vi "TXT to TDMS.vi"(8 "error in":errorcluster caption="エラー入力（エラーなし）", 11 "Original File name (TXT)":path) -> (0 "error out":errorcluster caption="エラー出力", 3 "Raw data Graph":dbl[](graph))   [LabVIEW 2018]
uses:
  <vilib>/Utility/file.llb/Read Delimited Spreadsheet (DBL).vi
panel:
  out "file or folder exists?":bool caption="既存するファイルまたはフォルダ?"
  out "all rows":dbl[][](array[numeric]) format="%0.3f"
  out "Create File name (TDMS)":path
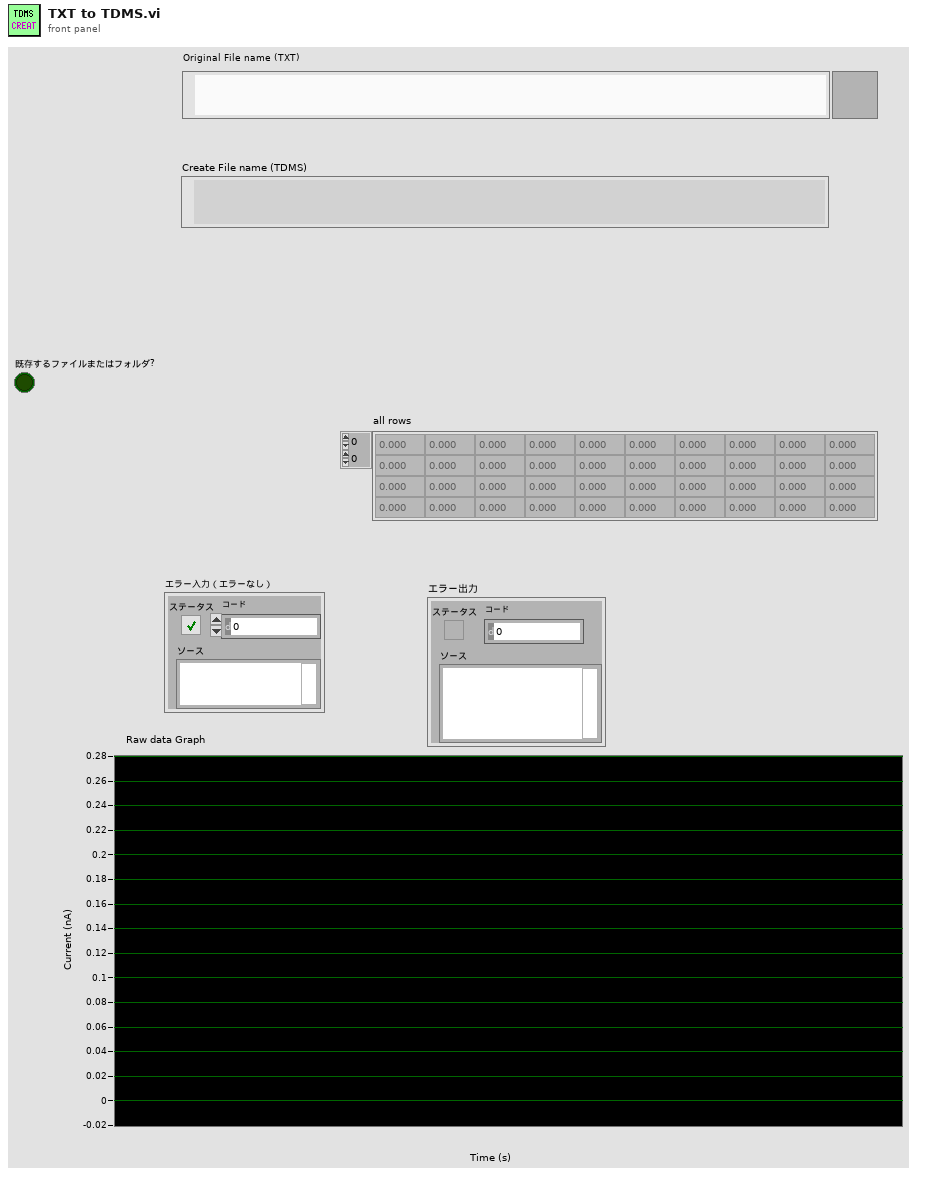
[diagram p1: front panel]
types:
  T1 = enum16{"open", "open or create", "create or replace", "create", "open (read-only)"}
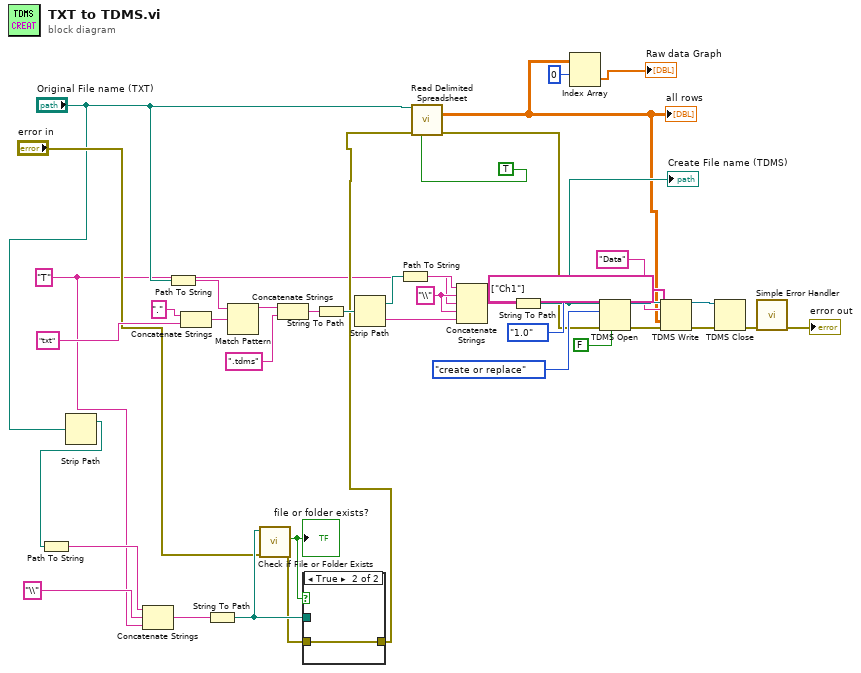
[diagram p0: block diagram]
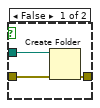
[diagram p2: hidden frame]
diagram:
  w4 = "T" ("Folder Name")
  w29 = "\\" ("文字列")
  n1 = Strip Path(path="Original File name (TXT)") -> (stripped path=w7:path)  [unwired: 1 out]
  n2 = Path To String(path=w7) -> (string=w6:string)
  n3 = Concatenate Strings(w6, "\\" ("文字列"), w4) -> (w12:string)
  n4 = Path To String(path="Original File name (TXT)") -> (string=w41:string)
  n5 = Concatenate Strings("." ("正規表現"), "txt" ("File Extention form")) -> (w36:string)
  n6 = String To Path(string=w12) -> (path=w13:path)
  n7 = Match Pattern(string=w41, regular expression=w36) -> (before substring=w40:string)  [unwired: 1 in, 3 out]
  n8 = call <vilib>:"Check if File or Folder Exists.vi"("error in (no error)"="error in", "path"=w13) -> ("error out"=w11:errorcluster, "file or folder exists?"=w14:bool)  [unwired: 7 in, 1 out]
  "file or folder exists?" <- w14
  n9 = Concatenate Strings(w40, ".tdms" ("文字列")) -> (w39:string)
  n10 = case shown="True" w14 {
    tunnel: w13 -> [w44 _]
    tunnel: w11 -> [w43 w45]
    tunnel: [w42 w45] -> w9
    frame False {
      n11 = Create Folder(path (use dialog)=w44, error in=w43) -> (error out=w42:errorcluster)  [unwired: 1 in, 2 out]
    }
    frame True {
    }
  }
  n12 = String To Path(string=w39) -> (path=w35:path)
  n13 = Strip Path(path=w35) -> (stripped path=w34:path, name=w30:string)
  n14 = Path To String(path=w34) -> (string=w33:string)
  n15 = call-poly <vilib>:"Read Delimited Spreadsheet.vi"("file path (dialog if empty)"="Original File name (TXT)", "error in (no error)"=w9, "transpose? (F)"=TRUE ("transpose (no:F)")) -> ("all rows"=w3:dbl[][], "error out"=w17:errorcluster)  [unwired: 7 in, 4 out]
  "all rows" <- w3
  n16 = Concatenate Strings(w33, w29, w4, w29, w30) -> (w32:string)
  n17 = String To Path(string=w32) -> (path=w19:path)
  "Create File name (TDMS)" <- w19
  n18 = Index Array(array=w3, index (row)=0 ("指標 （行）")) -> (element=→"Raw data Graph":dbl[])  [unwired: 1 in]
  n19 = TDMS Open(6:FALSE ("disable buffering (T)"), 7:enum16{"1.0", "2.0"}."1.0" ("file format version (2.0)"), 8:w17, 10:T1."create or replace" ("operation"), 11:w19) -> (0:w24:errorcluster, 3:w25:refnum<k34>)  [unwired: 2 in]
  n20 = TDMS Write(0:w25, 5:"Data" ("group name in (Untitled)"), 7:string[] ["Ch1"] ("チャンネル名入力（名称未設定）"), 9:w3, 11:w24) -> (4:w28:refnum<k34>, 15:w27:errorcluster)  [unwired: 1 in, 2 out]
  n21 = TDMS Close(8:w27, 11:w28) -> (0:w20:errorcluster)  [unwired: 1 out]
  n22 = call <vilib>:"Simple Error Handler.vi"("error in (no error)"=w20) -> ("error out"=→"error out":errorcluster)  [unwired: 1 in, 7 out]
